vi "_Load Markdown File.vi"(8 "Error In":errorcluster caption="error in (no error)", 11 "Path":path=path "D:/CSM Framework/Communicable-State-Machine/src/help/NEVSTOP/Communicable State Machine(CSM)") -> (0 "error out":errorcluster, 1 "Array 2":T1[](array[typedef]), 2 "Array":T2[](array[typedef]))   [LabVIEW 2017, in "csmdoc.lvlib"]
uses:
  csmdoc.lvlib
  _Typedef/DocElement.ctl
  _Typedef/DocNote.ctl
  _tool/_file/csm-file-support.lvlib
  Communicable State Machine.lvlib
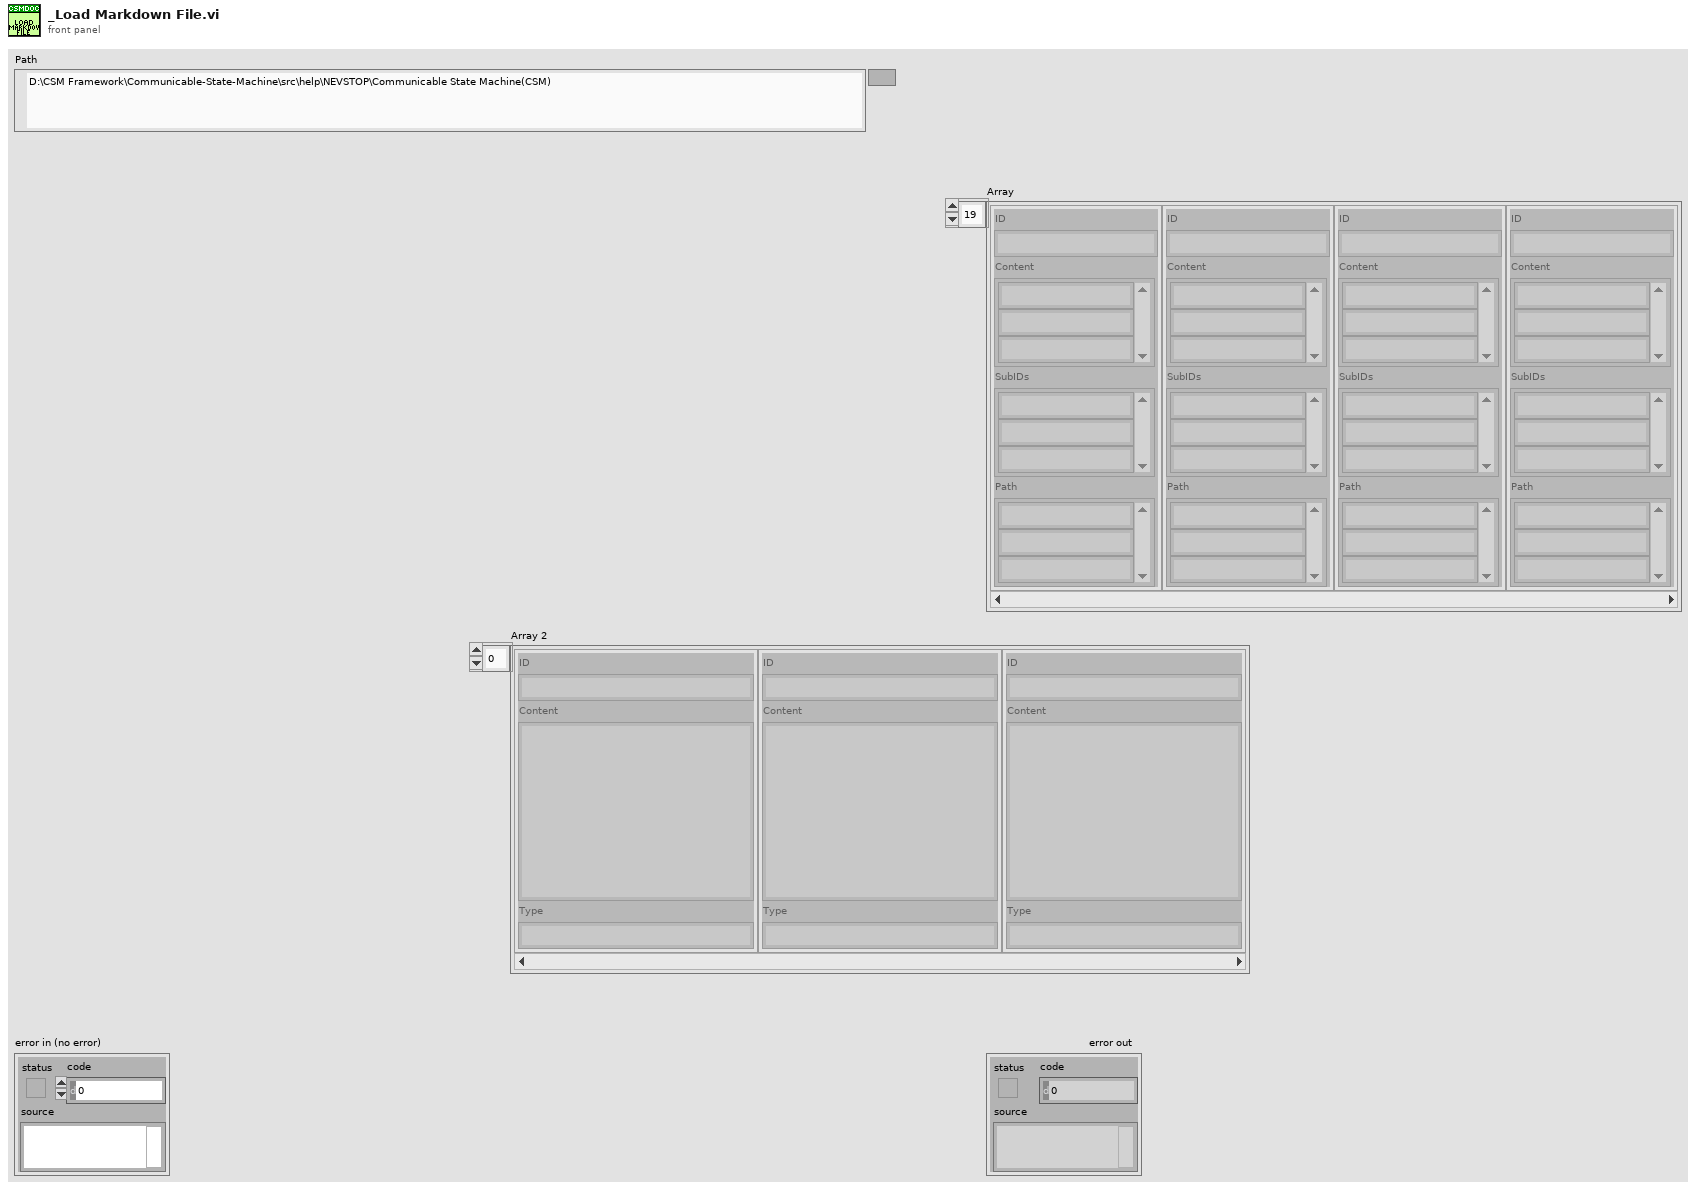
[diagram p1: front panel]
types:
  T1 = typedef "csmdoc.lvlib/DocNote.ctl" = cluster{"ID":string, "Content":string, "Type":string}
  T2 = typedef "csmdoc.lvlib/DocElement.ctl" = cluster{"ID":string, "Content":string[], "SubIDs":string[], "Path":string[]}
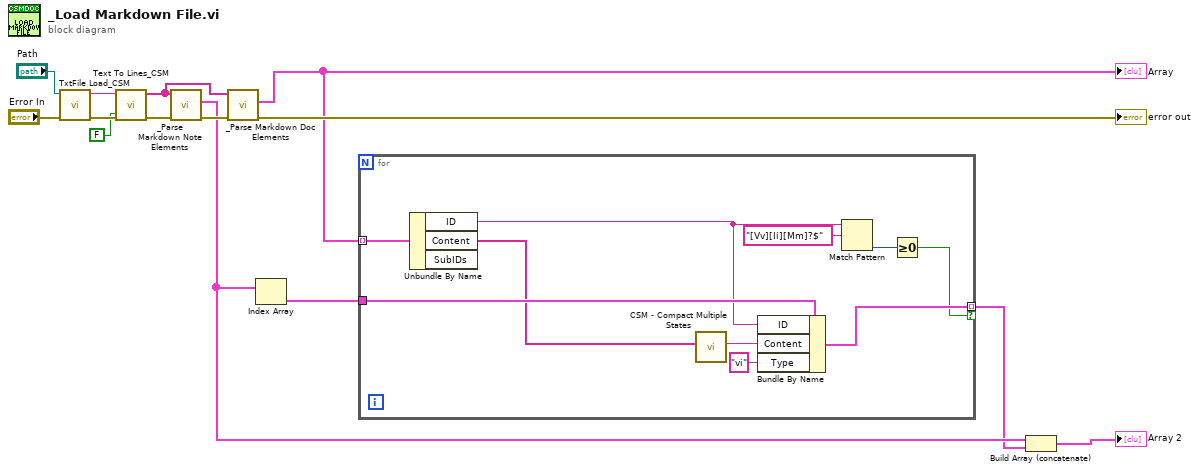
[diagram p0: block diagram]
diagram:
  n1 = call "TxtFile Load_CSM.vi"("error in (no error)"="Error In", "Path"="Path") -> ("error out"=w13:errorcluster, "Text"=w12:string)  [unwired: 8 in]
  n2 = call "Text To Lines_CSM.vi"("Remove Empty Lines? (T)"=FALSE ("Remove Empty Lines?(T)"), "error in (no error)"=w13, "String"=w12) -> ("error out"=w8:errorcluster, "Lines"=w9:string[])  [unwired: 7 in]
  n3 = call "_Parse Markdown Note Elements.vi"("Error in"=w8, "Lines"=w9) -> ("Error out"=w7:errorcluster, "Array"=w5:T1[])  [unwired: 7 in, 1 out]
  n4 = call "_Parse Markdown Doc Elements.vi"("Error in"=w7, "Lines"=w9) -> ("Error out"=→"error out":errorcluster, "Array"=w3:T2[])  [unwired: 7 in, 1 out]
  "Array" <- w3
  n5 = Index Array(array=w5) -> (element=w4:T1)  [unwired: 1 in]
  n6 = for {
    tunnel: w4 -> [w24]
    tunnel: w3 -> [w22] mode=indexing
    tunnel: [w19] -> w1 mode=indexing if=w15
    n7 = Unbundle By Name(w22) -> ("ID"=w18:string, "Content"=w21:string[])  [unwired: 1 out]
    n8 = call "CSM - Compact Multiple States.vi"("Multiple States"=w21) -> ("States"=w20:string)  [unwired: 9 in]
    n9 = Bundle By Name(cluster=w24, "ID"=w18, "Content"=w20, "Type"="vi") -> (w19:T1)
    n10 = Match Pattern(string=w18, regular expression="[Vv][Ii][Mm]?$") -> (offset past match=w16:i32)  [unwired: 1 in, 3 out]
    n11 = Greater Or Equal To 0?(x=w16) -> (x >= 0?=w15:bool)
  }
  n12 = Build Array (concatenate)(w5, w1) -> (→"Array 2":T1[])
